vi "Populate Type Definitions.vi"(8 "error in":errorcluster, 11 "G-CLI Runner in":refnum<class "Runner.lvclass">) -> (0 "error out":errorcluster, 3 "G-CLI Runner out":refnum<class "Runner.lvclass">)   [LabVIEW 2026, in "Runner.lvlib" / "Runner.lvclass"]
doc: "Create type definitions."
uses:
  Runner.lvclass
  Runner.lvclass/Runner.ctl
  Interfaces/ILogger/ILogger Messages/Log Msg/Log Msg.lvclass/Log Msg.ctl
  <vilib>/ActorFramework/Message Enqueuer/Message Enqueuer.lvclass/Message Enqueuer.ctl
  Classes/Type Definition/Type Definition.lvclass
  Classes/LabVIEW File/LabVIEW File.lvclass/LabVIEW File.ctl
  Classes/LabVIEW File/Write Name.vi
  <vilib>/ActorFramework/Message Enqueuer/Enqueue.vi
  Interfaces/ILogger/ILogger Messages/Log Msg/Log Msg.lvclass
  <vilib>/ActorFramework/Message Priority Queue/Priority Enqueue.vi
  Interfaces/ILV File Creator/ILV File Creator.lvclass
  Interfaces/IElement Manager/IElement Manager.lvclass
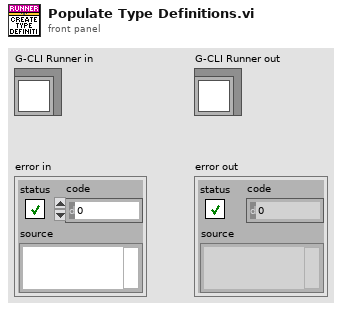
[diagram p1: front panel]
types:
  T1 = typedef "Type Definition--cluster.ctl" = cluster{"name":string, "fields":T2[]}
  T2 = typedef "Parameter--cluster.ctl" = cluster{"name":string, "data_type":string, "container":string, "dimensions":i32, "type_definition":string}
  T3 = typedef "Log Entry--cluster.ctl" = cluster{"Time":timestamp, "Message":string}
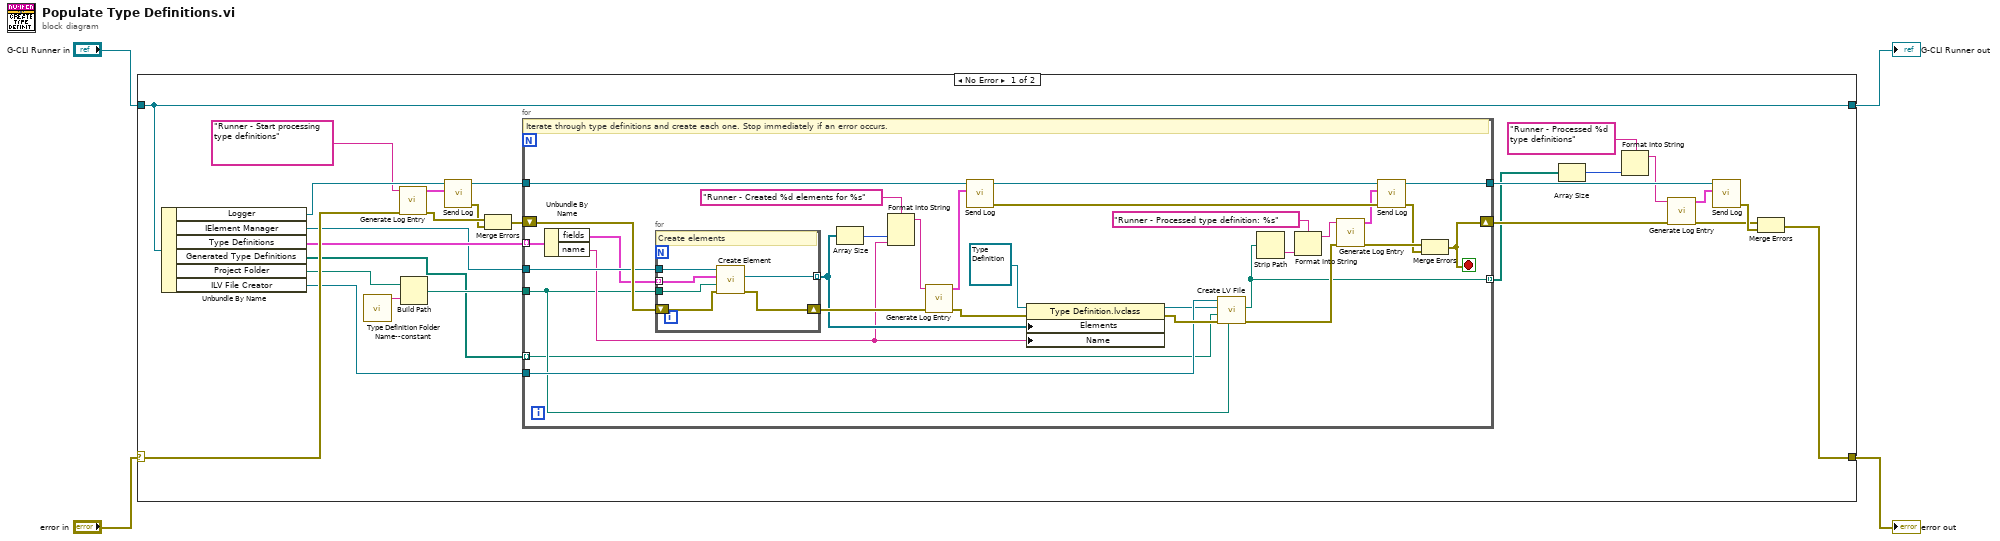
[diagram p0: block diagram]
diagram:
  n1 = case shown="No Error" "error in" {
    selector: "error in" -> [w23 w69]
    tunnel: [w27 w69] -> w4
    tunnel: "G-CLI Runner in" -> [w22 w68]
    tunnel: [w22 w68] -> w1
    frame No Error {
      n2 = Unbundle By Name(w22) -> ("Logger"=w16:refnum<class "Message Enqueuer.lvclass">, "IElement Manager"=w17:refnum<class "IElement Manager.lvclass">, "Type Definitions"=w21:T1[], "Generated Type Definitions"=w5:path[], "Project Folder"=w18:path, "ILV File Creator"=w12:refnum<class "ILV File Creator.lvclass">)
      n3 = call "Type Definition Folder Name--constant.vi"() -> ("Type Definition Folder Name"=w20:string)  [unwired: 11 in]
      n4 = call "Generate Log Entry.vi"("error in"=w23, "Message"="Runner - Start processing type definitions") -> ("error out"=w30:errorcluster, "Log Entry"=w14:T3)  [unwired: 8 in]
      n5 = Build Path(base path=w18, name or relative path=w20) -> (appended path=w19:path)
      n6 = call "Send Log.vi"("Log Entry"=w14, "Message Enqueuer"=w16) -> ("error out"=w28:errorcluster, "Message Enqueuer out"=w15:refnum<class "Message Enqueuer.lvclass">)  [unwired: 8 in]
      n7 = Merge Errors(w30, w28) -> (w29:errorcluster)
      n8 = for {
        tunnel: w21 -> [w52] mode=indexing
        tunnel: w19 -> [w32]
        shift-right: [w57] -> w25
        shift-left: w29 -> [w56]
        tunnel: w15 -> [w51]
        tunnel: [w36] -> w8 mode=indexing
        tunnel: w17 -> [w40]
        tunnel: w12 -> [w38]
        tunnel: [w34] -> w10
        tunnel: w5 -> [w31] mode=indexing
        stop <- w57 stop-if-true
        # "Iterate through type definitions and create each one. Stop immediately if an error occurs."
        n9 = Unbundle By Name(w52) -> ("fields"=w35:T2[], "name"=w33:string)
        n10 = for {
          tunnel: w40 -> [w65]
          tunnel: w35 -> [w64] mode=indexing
          tunnel: w32 -> [w63]
          tunnel: [w62] -> w39 mode=indexing
          shift-right: [w66] -> w53
          shift-left: w56 -> [w67]
          # "Create elements"
          n11 = call-dynamic "Create Element.vi"("error in"=w67, "Type Definitions Folder"=w63, "Parameter"=w64, "IElement Manager in"=w65) -> ("error out"=w66:errorcluster, "IElement"=w62:refnum<class "IElement.lvclass">)  [unwired: 5 in, 1 out]
        }
        n12 = Array Size(array=w39) -> (size(s)=w47:i32)
        n13 = Format Into String(format string="Runner - Created %d elements for %s", w47, w33) -> (resulting string=w48:string)  [unwired: 2 in, 1 out]
        n14 = call "Generate Log Entry.vi"("error in"=w53, "Message"=w48) -> ("error out"=w61:errorcluster, "Log Entry"=w46:T3)  [unwired: 8 in]
        n15 = call "Send Log.vi"("Log Entry"=w46, "Message Enqueuer"=w51) -> ("error out"=w60:errorcluster, "Message Enqueuer out"=w45:refnum<class "Message Enqueuer.lvclass">)  [unwired: 8 in]
        n16 = property on="Property Node" class="Type Definition.lvclass"(reference=refnum<class "Type Definition.lvclass"> refnum ("Type Definition.lvclass"), error in=w61, "Elements"=w39, "Name"=w33) -> (reference out=w37:refnum<class "Type Definition.lvclass">, error out=w55:errorcluster)
        n17 = call-dynamic "Create LV File.vi"("Output Folder"=w32, "error in"=w55, "Template"=w31, "ILabVIEW File"=w37, "ILV File Creator in"=w38) -> ("error out"=w54:errorcluster, "File Path"=w36:path)  [unwired: 4 in, 1 out]
        n18 = Strip Path(path=w36) -> (name=w41:string)  [unwired: 1 out]
        n19 = Format Into String(format string="Runner - Processed type definition: %s", w41) -> (resulting string=w43:string)  [unwired: 2 in, 1 out]
        n20 = call "Generate Log Entry.vi"("error in"=w54, "Message"=w43) -> ("error out"=w59:errorcluster, "Log Entry"=w42:T3)  [unwired: 8 in]
        n21 = call "Send Log.vi"("error in (no error)"=w60, "Log Entry"=w42, "Message Enqueuer"=w45) -> ("error out"=w58:errorcluster, "Message Enqueuer out"=w34:refnum<class "Message Enqueuer.lvclass">)  [unwired: 7 in]
        n22 = Merge Errors(w59, w58) -> (w57:errorcluster)
      }
      n23 = Array Size(array=w8) -> (size(s)=w7:i32)
      n24 = Format Into String(format string="Runner - Processed %d type definitions" ("Message"), w7) -> (resulting string=w6:string)  [unwired: 2 in, 1 out]
      n25 = call "Generate Log Entry.vi"("error in"=w25, "Message"=w6) -> ("error out"=w24:errorcluster, "Log Entry"=w11:T3)  [unwired: 8 in]
      n26 = call "Send Log.vi"("Log Entry"=w11, "Message Enqueuer"=w10) -> ("error out"=w26:errorcluster)  [unwired: 8 in, 1 out]
      n27 = Merge Errors(w24, w26) -> (w27:errorcluster)
    }
    frame Error {
      # "Pass error"
    }
  }
  "error out" <- w4
  "G-CLI Runner out" <- w1
